vi "MinMax Decimation.vi"(6 "Swap Axes (F)":bool, 10 "Params":T1, 11 "XY Data":cluster{"X":dbl[], "Y":dbl[]}[](array[cluster])) -> (3 "MinMax Data":cluster{dbl[], dbl[]}[](array[cluster]))   [LabVIEW 2020, in "VolatusGUIElements.lvlib"]
uses:
  VolatusGUIElements.lvlib
  Decimation Params.ctl
  First Last Samples.vi
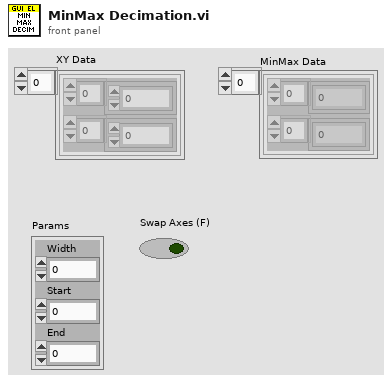
[diagram p1: front panel]
types:
  T1 = typedef "VolatusGUIElements.lvlib/Decimation Params.ctl" = cluster{"Width":i32, "Start":dbl, "End":dbl}
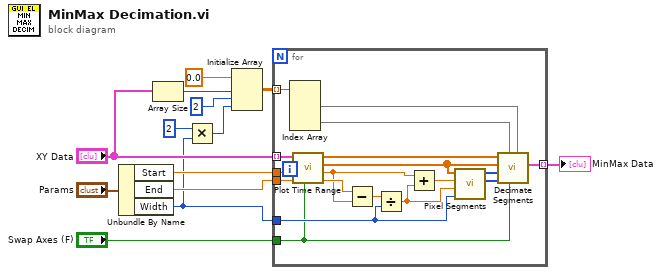
[diagram p0: block diagram]
diagram:
  n1 = Unbundle By Name("Params") -> ("Start"=w11:dbl, "End"=w10:dbl, "Width"=w5:i32)
  n2 = Array Size(array="XY Data") -> (size(s)=w7:i32)
  n3 = Multiply(x=2 ("y"), y=w5) -> (x*y=w4:i32)
  n4 = Initialize Array(0.0 ("element"), w7, 2 ("dimension size"), w4) -> (w3:dbl[][][])
  n5 = for {
    tunnel: w11 -> [w24]
    tunnel: w10 -> [w25]
    tunnel: "XY Data" -> [w31] mode=indexing
    tunnel: w5 -> [w22]
    tunnel: [w26] -> w12 mode=indexing
    tunnel: w3 -> [w17] mode=indexing
    tunnel: "Swap Axes (F)" -> [w14]
    n6 = Index Array(array=w17) -> (element #1=w15:dbl[], element #2=w16:dbl[])  [unwired: 4 in]
    n7 = call "Plot Time Range.vi"("Swap Axes"=w14, "End"=w25, "Start"=w24, "Plot Data"=w31) -> ("Actual End"=w19:dbl, "Actual Start"=w18:dbl, "Independent"=w29:dbl[], "Dependent"=w30:dbl[])  [unwired: 4 in]
    n8 = Subtract(x=w19, y=w18) -> (x-y=w23:dbl)
    n9 = Divide(x=w23, y=w22) -> (x/y=w20:dbl)
    n10 = Add(x=w18, y=w20) -> (x+y=w21:dbl)
    n11 = call "Pixel Segments.vi"("# px"=w22, "ds / px"=w20, "End of First px"=w21, "Independent"=w29) -> ("px Lengths"=w27:i32[], "px Starts"=w28:i32[])  [unwired: 6 in]
    n12 = call "Decimate Segments.vi"("Y Buffer"=w15, "Swap Axes"=w14, "X Buffer"=w16, "px Lengths"=w27, "px Starts"=w28, "Independent"=w29, "Dependent"=w30) -> ("Decimated Data"=w26:cluster{"X":dbl[], "Y":dbl[]})  [unwired: 4 in]
  }
  "MinMax Data" <- w12
